vi "ZM-CM-writePrelaunchSettings.vi"(8 "error in (no error)":errorcluster, 10 "settings":T1, 11 "ZM-CM-communication_manager in":refnum<class "ZM-CM-communication_manager.lvclass">) -> (0 "error out":errorcluster, 3 "ZM-CM-communication_manager out":refnum<class "ZM-CM-communication_manager.lvclass">)   [LabVIEW 2020, in "ZM-CM-communication_manager.lvlib" / "ZM-CM-communication_manager.lvclass"]
doc: "Public custom accessor: writes the pre-launch settings. The caller fills ZM-CM-PRELAUNCH_SETTINGS (the protocol) and then launches the actor."
uses:
  ZM-CM-communication_manager.lvclass
  protocol/ZM-CP-communication_protocol/ZM-CP-communication_protocol/ZM-CP-communication_protocol.lvclass
  ZM-CM-communication_manager.lvclass/ZM-CM-communication_manager.ctl
  ZM-CM-PRELAUNCH_SETTINGS.ctl
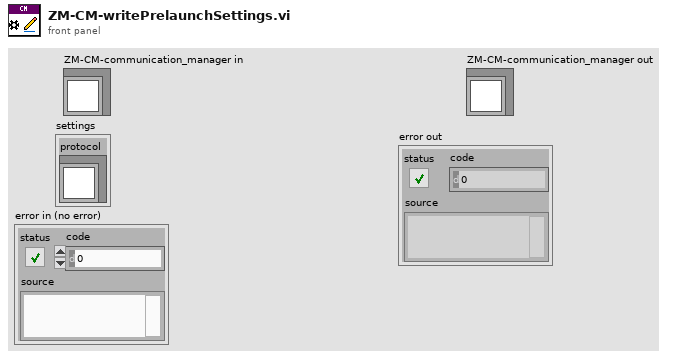
[diagram p1: front panel]
types:
  T1 = typedef "ZM-CM-communication_manager.lvlib/ZM-CM-communication_manager.lvclass/ZM-CM-PRELAUNCH_SETTINGS.ctl" = cluster{"protocol":refnum<class "ZM-CP-communication_protocol.lvclass">}
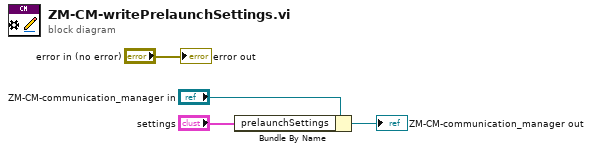
[diagram p0: block diagram]
diagram:
  n1 = Bundle By Name(cluster="ZM-CM-communication_manager in", "prelaunchSettings"="settings") -> (→"ZM-CM-communication_manager out":refnum<class "ZM-CM-communication_manager.lvclass">)
  "error out" <- "error in (no error)"
